vi "Add Button.vi"(8 "error in (no error)":errorcluster, 10 "button":refnum<k24>, 11 "reference":refnum<k24>) -> (0 "error out":errorcluster, 3 "reference out":refnum<k24>)   [LabVIEW 2026, in "ToastNotification.lvlib" / "Toast Native.lvlib"]
doc: "Native AddButton call on a borrowed ToastContentBuilder using a borrowed ToastButton. reference out aliases the builder. This VI does not close either input handle. The caller that acquired the button handle must release it after use; adding the managed button to the builder is not a second LabVIEW handle acquisition."
uses:
  Toast Native.lvlib
  C:/Users/loicw/Documents/LabVIEW/ToastNotifications/Sources/bins/Microsoft.Toolkit.Uwp.Notifications.dll
  bins/Microsoft.Toolkit.Uwp.Notifications.dll
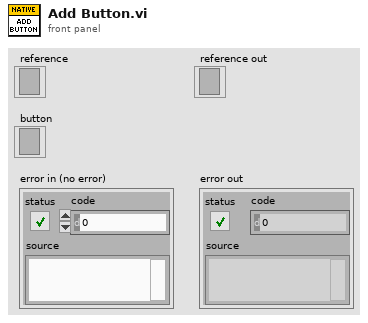
[diagram p1: front panel]
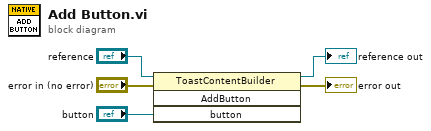
[diagram p0: block diagram]
diagram:
  n1 = invoke class="ToastContentBuilder" method="AddButton"(reference="reference", error in="error in (no error)", "button"="button") -> (reference out=→"reference out":refnum<k24>, error out=→"error out":errorcluster)  [unwired: 1 in, 2 out]
